vi "CSE Callback DlgDbg - Reinit Variables.vi"(8 "error in":errorcluster, 9 "action":T2(ring), 11 "VC Handle":T1=-1) -> (0 "error out":errorcluster, 3 "dup VC Handle":T1=-1)   [LabVIEW 2021]
doc: "::: CalcExpress Toolkit :::\nCopyright (c) 2000-2026 Konstantin Shifershteyn. All rights reserved."
uses:
  vi.lib/addons/CalcExpress/cetypes.llb/VarMan Variable Context Handle.ctl
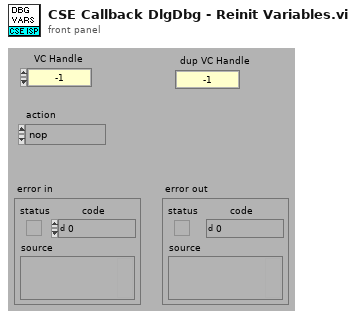
[diagram p1: front panel]
types:
  T1 = typedef "VarMan Variable Context Handle.ctl" = i32
  T2 = enum32{"nop", "save info", "restore info", "remove info"}
  T3 = enum16{"create", "destroy", "set value", "get value"}
  T4 = typedef "VarMan Variable Info Cluster.ctl" = cluster{"name":string, "alias":string, "type":u32, "history":bool}
  T5 = cluster{"alias":string, "dup name_spec":string, "flattened value out":string, "var type out":u32}
  T6 = cluster{cluster{"alias":string, "dup name_spec":string, "flattened value out":string, "var type out":u32}[]}
  T7 = cluster{cluster{"alias":string, "dup name_spec":string, "flattened value out":string, "var type out":u32}[]}[]
  T8 = cluster{"alias":string, "dup name_spec":string, "flattened value out":string, "var type out":u32}[]
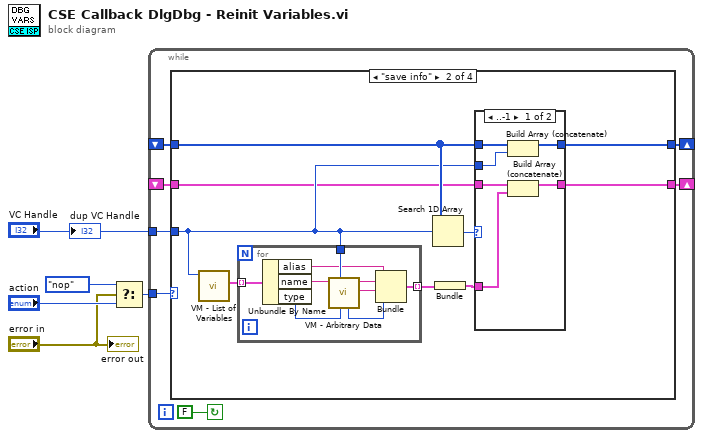
[diagram p0: block diagram]
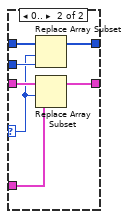
[diagram p3: hidden frame]
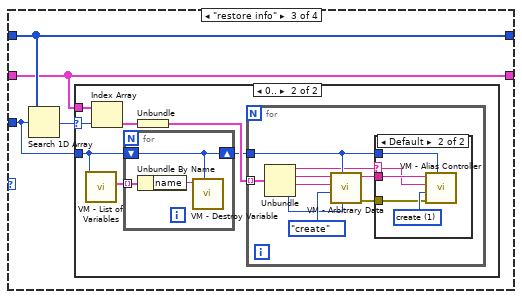
[diagram p4: hidden frame]
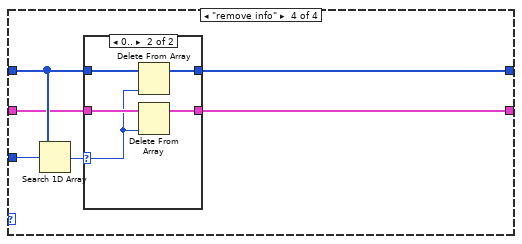
[diagram p7: hidden frame]
diagram:
  n1 = Select(t=T2."nop", s="error in", f="action") -> (s? t:f=w3:T2)
  n2 = while {
    shift-right: [w9] -> _
    shift-left: _ -> [w10]
    shift-right: [w7] -> _
    shift-left: _ -> [w8]
    tunnel: w3 -> [w12]
    tunnel: "VC Handle" -> [w11]
    stop <- FALSE continue-if-true
    n3 = case shown="\"save info\"" w12 {
      tunnel: w11 -> [_ w19 w47 w76]
      tunnel: w10 -> [w14 w21 w48 w78]
      tunnel: [w14 w20 w48 w77] -> w9
      tunnel: w8 -> [w13 w18 w46 w75]
      tunnel: [w13 w17 w46 w74] -> w7
      frame "nop" {
      }
      frame "save info" {
        n4 = call "VM - List of Variables.vi"("VC Handle"=w19) -> ("variables info"=w23:T4[])  [unwired: 6 in, 2 out]
        n5 = for {
          tunnel: w23 -> [w45] mode=indexing
          tunnel: [w40] -> w16 mode=indexing
          tunnel: w19 -> [w39]
          n6 = Unbundle By Name(w45) -> ("alias"=w37:string, "name"=w44:string, "type"=w38:u32)
          n7 = call "VM - Arbitrary Data.vi"("var type"=w38, "VC Handle"=w39, "name_spec"=w44) -> ("flattened value out"=w42:string, "dup name_spec"=w43:string, "var type out"=w41:u32)  [unwired: 3 in, 3 out]
          n8 = Bundle("alias"=w37, "dup name_spec"=w43, "flattened value out"=w42, "var type out"=w41) -> (w40:T5)  [unwired: 1 in]
        }
        n9 = Search 1D Array(1D array=w21, element=w19) -> (index of element=w22:i32)  [unwired: 1 in]
        n10 = Bundle(w16) -> (w15:T6)  [unwired: 1 in]
        n11 = case shown="..-1" w22 {
          selector: w22 -> [_ w31]
          tunnel: w21 -> [w29 w36]
          tunnel: [w28 w30] -> w20
          tunnel: w19 -> [w27 w35]
          tunnel: w18 -> [w26 w34]
          tunnel: [w25 w33] -> w17
          tunnel: w15 -> [w24 w32]
          frame ..-1 {
            n12 = Build Array (concatenate)(w29, w27) -> (w28:T1[])
            n13 = Build Array (concatenate)(w26, w24) -> (w25:T7)
          }
          frame 0.. {
            n14 = Replace Array Subset(array=w36, new element=w35, index=w31) -> (w30:T1[])
            n15 = Replace Array Subset(array=w34, new element=w32, index=w31) -> (w33:T7)
          }
        }
      }
      frame "restore info" {
        n16 = Search 1D Array(1D array=w48, element=w47) -> (index of element=w49:i32)  [unwired: 1 in]
        n17 = case shown="0.." w49 {
          selector: w49 -> [_ w55]
          tunnel: w47 -> [_ w51]
          tunnel: w46 -> [_ w54]
          frame ..-1 {
          }
          frame 0.. {
            n18 = call "VM - List of Variables.vi"("VC Handle"=w51) -> ("variables info"=w56:T4[])  [unwired: 6 in, 2 out]
            n19 = Index Array(array=w54, index=w55) -> (element=w53:T6)
            n20 = for {
              tunnel: w56 -> [w73] mode=indexing
              shift-right: [w71] -> w50
              shift-left: w51 -> [w71]
              n21 = Unbundle By Name(w73) -> ("name"=w72:string)
              n22 = call "VM - Destroy Variable.vi"("VC Handle"=w71, "name_spec"=w72) -> ()  [unwired: 6 in, 4 out]
            }
            n23 = Unbundle(w53) -> (w52:T8)
            n24 = for {
              tunnel: w52 -> [w65] mode=indexing
              tunnel: w50 -> [w62]
              n25 = Unbundle(w65) -> ("alias"=w60:string, "dup name_spec"=w59:string, "flattened value out"=w58:string, "var type out"=w57:u32)
              n26 = call "VM - Arbitrary Data.vi"("var type"=w57, "VC Handle"=w62, "cmd"=T3."create", "flattened value"=w58, "name_spec"=w59) -> ("error out"=w61:errorcluster, "dup name_spec"=w63:string)  [unwired: 1 in, 4 out]
              n27 = case shown="Default" w60 {
                selector: w60 -> [_ w66]
                tunnel: w63 -> [_ w69]
                tunnel: w62 -> [_ w68]
                tunnel: w61 -> [_ w67]
                frame "" {
                }
                frame Default {
                  w70 = u32 1 items=["nop", "create", "create or rename", "dispose"] ("action")
                  n28 = call "VM - Alias Controller.vi"("VC Handle"=w68, "error in"=w67, "action"=w70, "alias"=w66, "name_spec"=w69) -> ()  [unwired: 3 in, 4 out]
                }
              }
            }
          }
        }
      }
      frame "remove info" {
        n29 = Search 1D Array(1D array=w78, element=w76) -> (index of element=w79:i32)  [unwired: 1 in]
        n30 = case shown="0.." w79 {
          selector: w79 -> [_ w82]
          tunnel: w78 -> [w81 w86]
          tunnel: [w81 w83] -> w77
          tunnel: w75 -> [w80 w85]
          tunnel: [w80 w84] -> w74
          frame ..-1 {
          }
          frame 0.. {
            n31 = Delete From Array(array=w86, index=w82) -> (array with subset deleted=w83:T1[])  [unwired: 1 in, 1 out]
            n32 = Delete From Array(array=w85, index=w82) -> (array with subset deleted=w84:T7)  [unwired: 1 in, 1 out]
          }
        }
      }
    }
  }
  "dup VC Handle" <- "VC Handle"
  "error out" <- "error in"
